vi "serial.vi"() -> ()   [LabVIEW 2019]
uses:
  <vilib>/Instr/_visa.llb/VISA Configure Serial Port (Instr).vi
panel:
  out "SUICHE":bool
  out "TEMPERATURA":dbl(slide) scale=0.0..100.0
  out "read buffer":string
  in  "PARAR":bool
  in  "PUERTO":refnum<visa-resource-name>="COM4"
  in  "Izquierda":bool
  in  "Derecha":bool
  in  "VELOCIDAD":dbl(knob) scale=0.0..100.0
  in  "LED2":bool
  in  "LED1":bool
  in  "stop":bool
  # "GIRO"
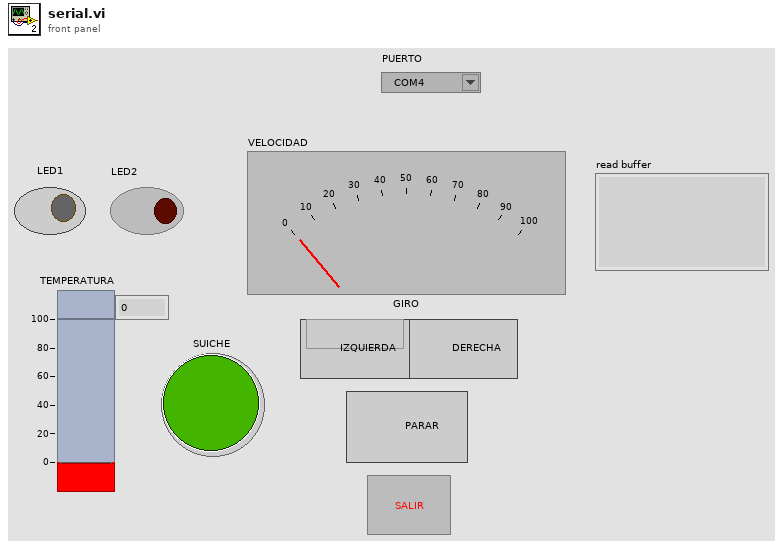
[diagram p1: front panel]
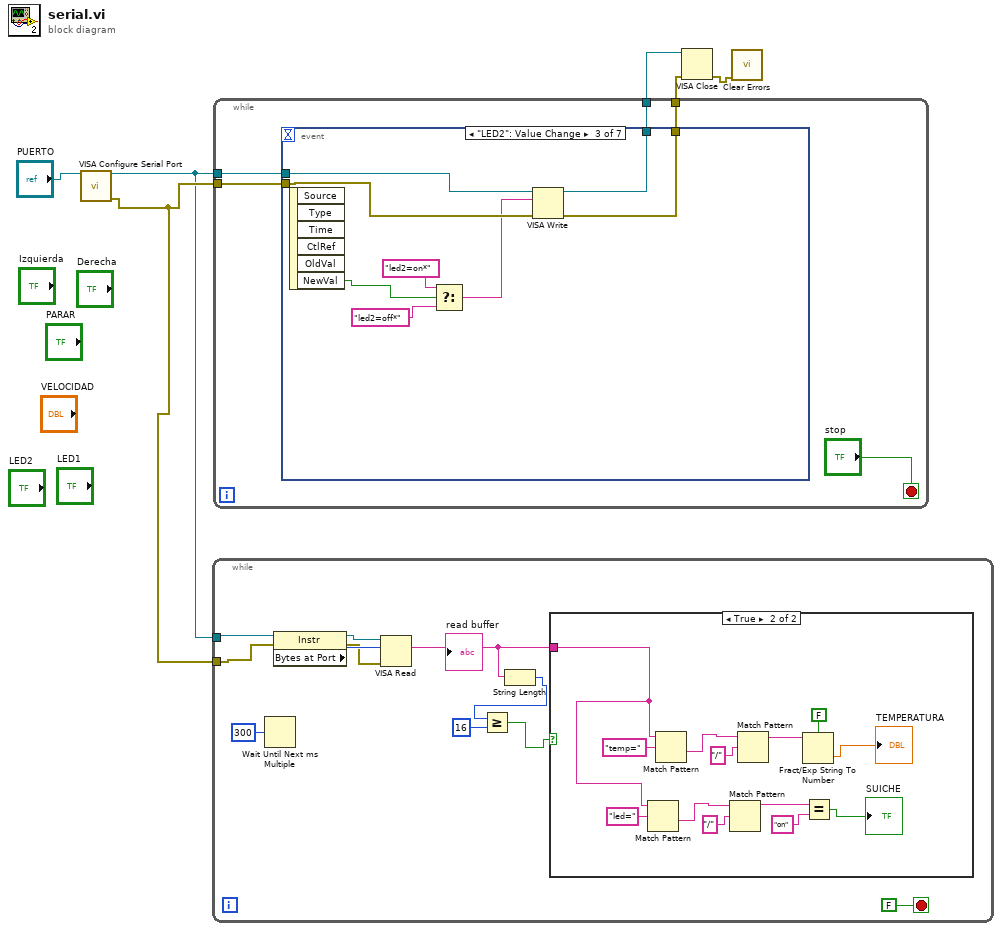
[diagram p0: block diagram]
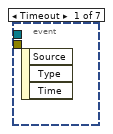
[diagram p3: hidden frame]
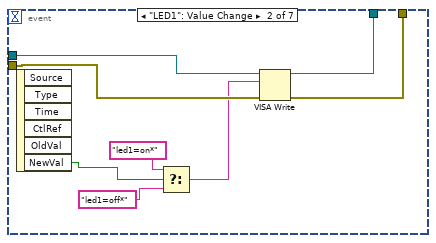
[diagram p4: hidden frame]
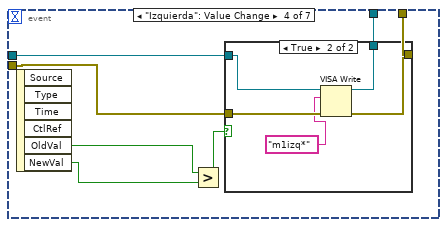
[diagram p5: hidden frame]
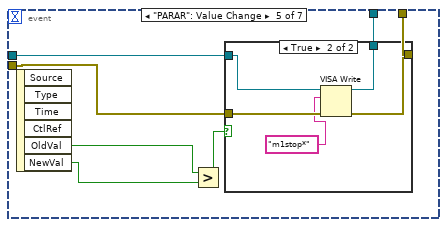
[diagram p7: hidden frame]
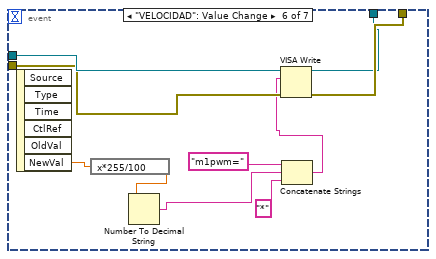
[diagram p9: hidden frame]
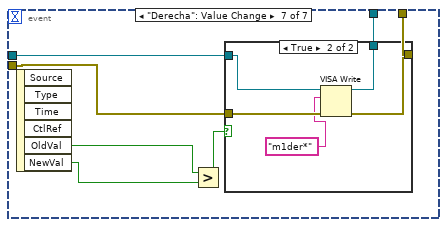
[diagram p10: hidden frame]
diagram:
  n1 = call-poly "VISA Configure Serial Port"("VISA resource name"="PUERTO") -> ("VISA resource name out"=w1:refnum<visa-resource-name>, "error out"=w2:errorcluster)  [unwired: 13 in]
  n2 = while {
    tunnel: w2 -> [w12]
    tunnel: w1 -> [w13]
    stop <- FALSE stop-if-true
    n3 = Wait Until Next ms Multiple(millisecond multiple=u32 300) -> ()  [unwired: 1 out]
    n4 = property class="Instr"(reference=w13, error in=w12) -> (reference out=w15:refnum<visa-resource-name>, error out=w14:errorcluster, "Bytes at Port"=w16:u32)
    n5 = VISA Read(VISA resource name=w15, byte count=w16, error in (no error)=w14) -> (read buffer=w10:string)  [unwired: 3 out]
    "read buffer" <- w10
    n6 = String Length(string=w10) -> (length=w9:i32)
    n7 = Greater Or Equal?(x=w9, y=16) -> (x >= y?=w7:bool)
    n8 = case shown="True" w7 {
      tunnel: w10 -> [_ w18]
      frame False {
      }
      frame True {
        n9 = Match Pattern(string=w18, regular expression="led=") -> (after substring=w23:string)  [unwired: 1 in, 3 out]
        n10 = Match Pattern(string=w18, regular expression="temp=") -> (after substring=w29:string)  [unwired: 1 in, 3 out]
        n11 = Match Pattern(string=w23, regular expression="/") -> (before substring=w21:string)  [unwired: 1 in, 3 out]
        n12 = Match Pattern(string=w29, regular expression="/") -> (before substring=w27:string)  [unwired: 1 in, 3 out]
        n13 = Fract/Exp String To Number(use system decimal point (T)=FALSE, string=w27) -> (number=→"TEMPERATURA":dbl)  [unwired: 2 in, 1 out]
        n14 = Equal?(x=w21, y="on") -> (x = y?=→"SUICHE":bool)
      }
    }
  }
  n15 = while {
    tunnel: w1 -> [w34]
    tunnel: w2 -> [w33]
    tunnel: [w32] -> w5
    tunnel: [w31] -> w4
    stop <- "stop" stop-if-true
    n16 = event shown="[2] \"LED2\": Value Change" {
      selector: _ -> [_ _ _ _ _ _ _]
      dyn-events: _ -> [_ _ _ _ _ _ _]
      timeout: _ -> [_ _ _ _ _ _ _]
      tunnel: w34 -> [_ w43 w51 w58 w70 w85 w92]
      tunnel: w33 -> [_ w42 w50 w57 w69 w84 w91]
      tunnel: [_ w37 w45 w56 w68 w82 w90] -> w32
      tunnel: [_ w36 w44 w55 w67 w83 w89] -> w31
      event Timeout {
        n17 = event-data() -> ()  [unwired: 1 in, 3 out]
      }
      event "LED1": Value Change {
        n18 = event-data() -> ("NewVal"=w41:bool)  [unwired: 1 in, 5 out]
        n19 = Select(t="led1=on*", s=w41, f="led1=off*") -> (s? t:f=w38:string)
        n20 = VISA Write(VISA resource name=w43, write buffer=w38, error in (no error)=w42) -> (VISA resource name out=w37:refnum<visa-resource-name>, error out=w36:errorcluster)  [unwired: 1 out]
      }
      event "LED2": Value Change {
        n21 = event-data() -> ("NewVal"=w49:bool)  [unwired: 1 in, 5 out]
        n22 = Select(t="led2=on*", s=w49, f="led2=off*") -> (s? t:f=w46:string)
        n23 = VISA Write(VISA resource name=w51, write buffer=w46, error in (no error)=w50) -> (VISA resource name out=w45:refnum<visa-resource-name>, error out=w44:errorcluster)  [unwired: 1 out]
      }
      event "Izquierda": Value Change {
        n24 = event-data() -> ("OldVal"=w54:bool, "NewVal"=w53:bool)  [unwired: 1 in, 4 out]
        n25 = Greater?(x=w54, y=w53) -> (0:w52:bool)
        n26 = case shown="True" w52 {
          tunnel: w58 -> [_ w63]
          tunnel: w57 -> [_ w62]
          tunnel: [_ w61] -> w56
          tunnel: [_ w60] -> w55
          frame False {
          }
          frame True {
            n27 = VISA Write(VISA resource name=w63, write buffer="m1izq*", error in (no error)=w62) -> (VISA resource name out=w61:refnum<visa-resource-name>, error out=w60:errorcluster)  [unwired: 1 out]
          }
        }
      }
      event "PARAR": Value Change {
        n28 = event-data() -> ("OldVal"=w66:bool, "NewVal"=w65:bool)  [unwired: 1 in, 4 out]
        n29 = Greater?(x=w66, y=w65) -> (0:w64:bool)
        n30 = case shown="True" w64 {
          tunnel: w70 -> [_ w75]
          tunnel: w69 -> [_ w74]
          tunnel: [_ w73] -> w68
          tunnel: [_ w72] -> w67
          frame False {
          }
          frame True {
            n31 = VISA Write(VISA resource name=w75, write buffer="m1stop*", error in (no error)=w74) -> (VISA resource name out=w73:refnum<visa-resource-name>, error out=w72:errorcluster)  [unwired: 1 out]
          }
        }
      }
      event "VELOCIDAD": Value Change {
        n32 = event-data() -> ("NewVal"=w77:dbl)  [unwired: 1 in, 5 out]
        n33 = expression code="x*255/100"(w77) -> (w76:dbl)
        n34 = Number To Decimal String(number=w76) -> (decimal integer string=w80:string)  [unwired: 1 in]
        n35 = Concatenate Strings("m1pwm=" ("string"), w80, "*" ("string")) -> (w78:string)
        n36 = VISA Write(VISA resource name=w85, write buffer=w78, error in (no error)=w84) -> (VISA resource name out=w82:refnum<visa-resource-name>, error out=w83:errorcluster)  [unwired: 1 out]
      }
      event "Derecha": Value Change {
        n37 = event-data() -> ("OldVal"=w88:bool, "NewVal"=w87:bool)  [unwired: 1 in, 4 out]
        n38 = Greater?(x=w88, y=w87) -> (0:w86:bool)
        n39 = case shown="True" w86 {
          tunnel: w92 -> [_ w97]
          tunnel: w91 -> [_ w96]
          tunnel: [_ w95] -> w90
          tunnel: [_ w94] -> w89
          frame False {
          }
          frame True {
            n40 = VISA Write(VISA resource name=w97, write buffer="m1der*", error in (no error)=w96) -> (VISA resource name out=w95:refnum<visa-resource-name>, error out=w94:errorcluster)  [unwired: 1 out]
          }
        }
      }
    }
  }
  n41 = VISA Close(VISA resource name=w5, error in (no error)=w4) -> (error out=w3:errorcluster)
  n42 = call <vilib>:"Clear Errors.vi"("error in (no error)"=w3) -> ()  [unwired: 5 in, 2 out]
